vi "PrimaryProviderExample_CreateNewWizard_IncludeItem.vi"(11 "Wizard":T1) -> (3 "Include me":bool)   [LabVIEW 2027]
uses:
  <resource>/Framework/Providers/API/ItemRef.ctl
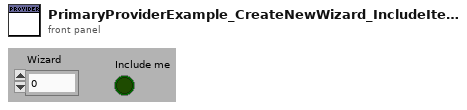
[diagram p1: front panel]
types:
  T1 = typedef "ItemRef.ctl" = u64
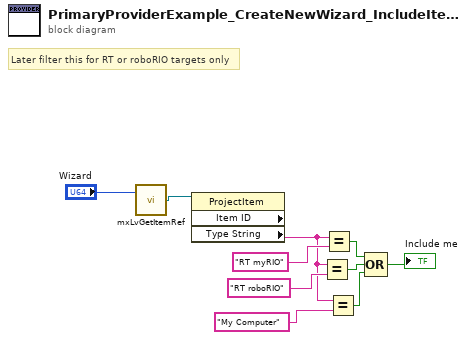
[diagram p0: block diagram]
diagram:
  # "Later filter this for RT or roboRIO targets only"
  n1 = call <resource>:"mxLvGetItemRef.vi"("Item"="Wizard") -> ("Item Refnum"=w9:refnum<vi>)  [unwired: 1 in, 2 out]
  n2 = property class="ProjectItem" props=["Item ID", "Type String"](reference=w9) -> ("Type String"=w2:string)  [unwired: 1 in, 3 out]
  n3 = Equal?(x=w2, y="RT roboRIO" ("message")) -> (x = y?=w4:bool)
  n4 = Equal?(x=w2, y="RT myRIO" ("message")) -> (x = y?=w6:bool)
  n5 = Equal?(x=w2, y="My Computer" ("Type String")) -> (x = y?=w3:bool)
  n6 = Compound Arithmetic op=OR(w6, w4, w3) -> (→"Include me":bool)
